vi "Registry_Resolve.vi"(8 "error in (no error)":errorcluster={"status"=FALSE, "code"=0, "source"="\"\""}, 10 "definitions/results":string, 11 "Reference ID":string) -> (0 "error out":errorcluster={"status"=FALSE, "code"=0, "source"="\"\""}, 2 "status ok":bool, 3 "Definition and current value":string)   [LabVIEW 2026]
doc: "INTENT: Map parameter or result ID. LOGIC: Resolve logical ID to known source; return explicit lookup error."
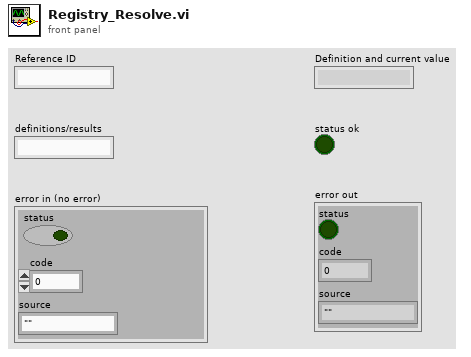
[diagram p1: front panel]
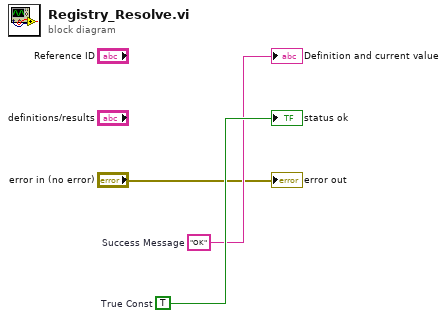
[diagram p0: block diagram]
diagram:
  w3 = TRUE  # True Const
  w2 = "OK"  # Success Message
  "Definition and current value" <- w2
  "status ok" <- w3
  "error out" <- "error in (no error)"
